vi "takeuchi_2026_01.vi"() -> ()   [LabVIEW 2026]
uses:
  <vilib>/Utility/file.llb/Write Delimited Spreadsheet (DBL).vi
panel:
  out "SOV?":string
  out "Specified voltage":string
  in  "Boolean":bool
  in  "delay time (s)":dbl
  out "Remaining time (s)":i32
  out "XY Graph":cluster{dbl[], dbl[]}(graph)
  in  "Start Voltage(V)":dbl
  in  "Goal Voltage(V)":dbl
  in  "Step (mV)":dbl
  in  "base path":path
  in  "File name":string
  # "temp"
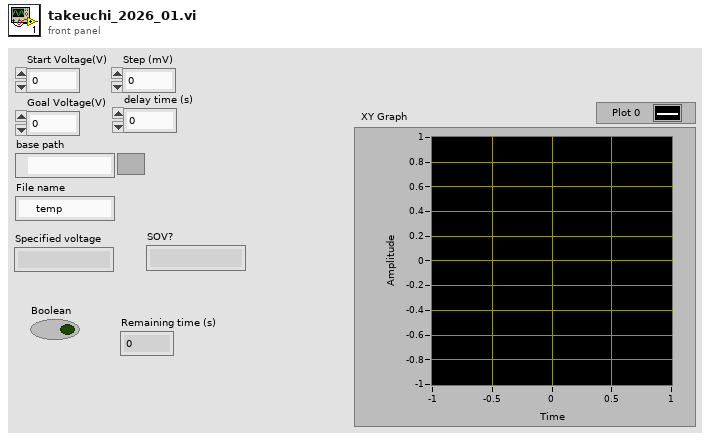
[diagram p1: front panel]
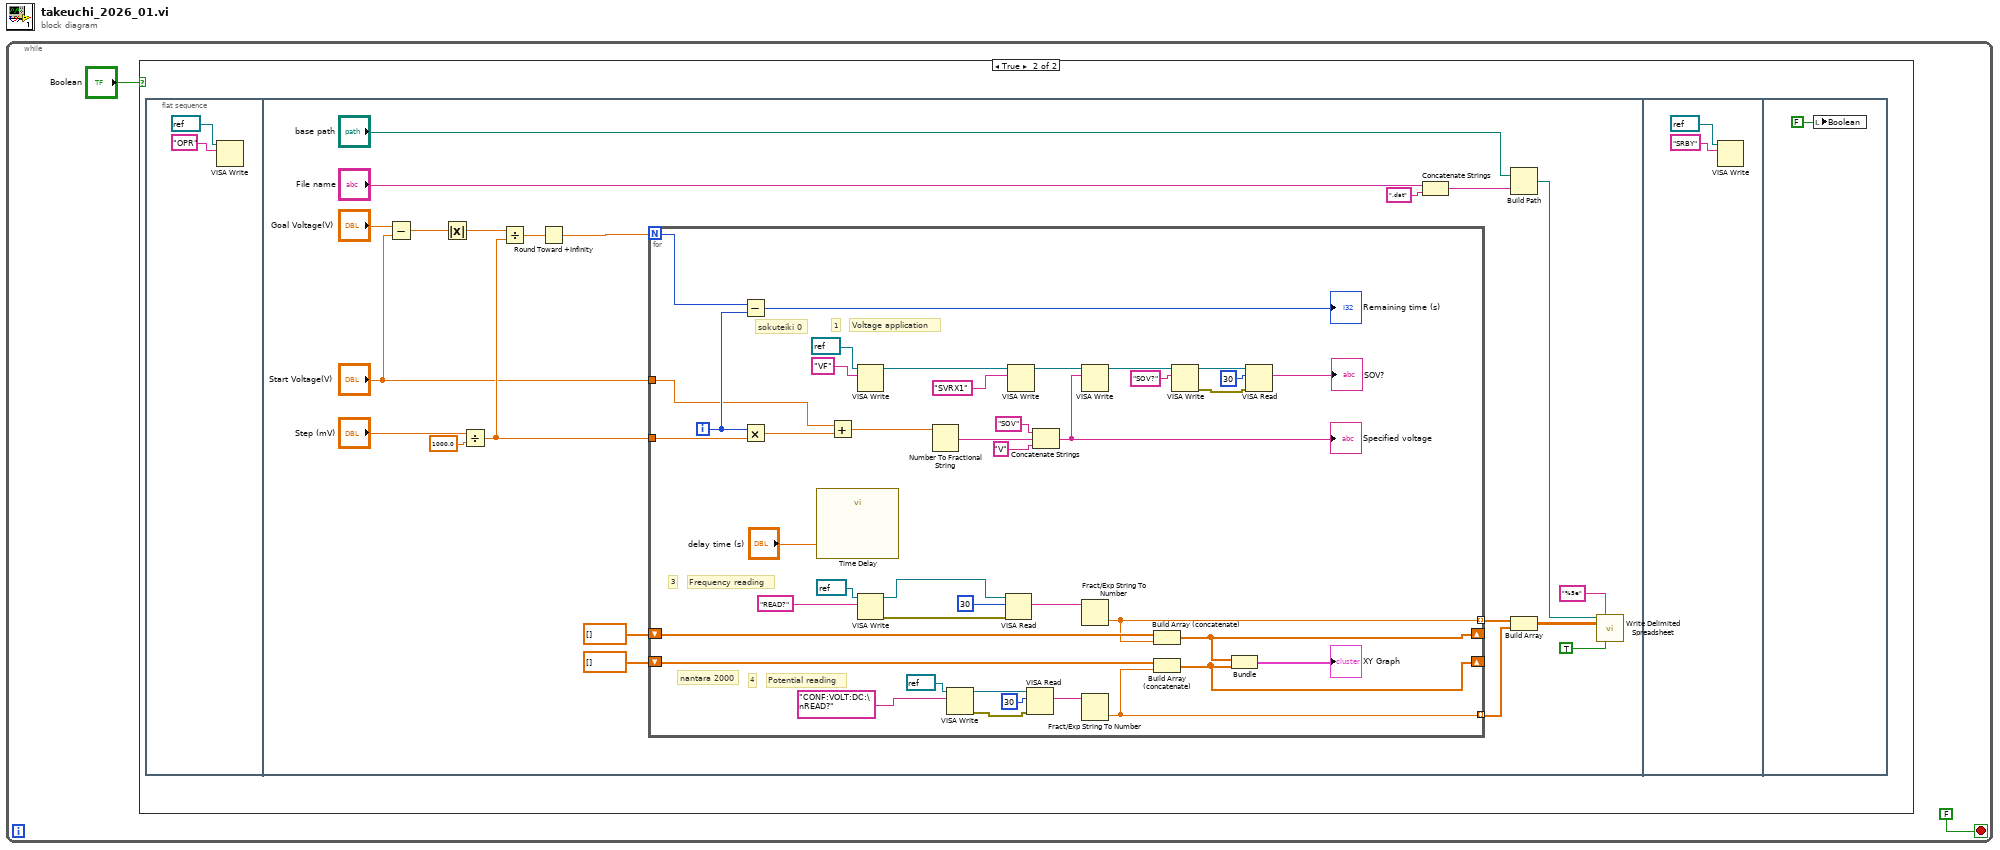
[diagram p0: block diagram]
diagram:
  n1 = while {
    stop <- FALSE stop-if-true
    n2 = case shown="True" "Boolean" {
      frame False {
      }
      frame True {
        n3 = flat-sequence {
          frame #0 {
            n4 = VISA Write(VISA resource name=refnum<visa-resource-name> refnum, write buffer="OPR") -> ()  [unwired: 1 in, 3 out]
          }
          frame #1 {
            n5 = Subtract(x="Goal Voltage(V)", y="Start Voltage(V)") -> (x-y=w24:dbl)
            n6 = Absolute Value(x=w24) -> (abs(x)=w23:dbl)
            n7 = Divide(x="Step (mV)", y=1000.0) -> (x/y=w18:dbl)
            n8 = Divide(x=w23, y=w18) -> (x/y=w20:dbl)
            n9 = Round Toward +Infinity(x=w20) -> (ceil(x): smallest int >= x=w19:dbl)
            n10 = for {
              N: w19 -> [w67]
              tunnel: w18 -> [w65]
              tunnel: "Start Voltage(V)" -> [w63]
              shift-right: [w44] -> _
              shift-left: dbl[] [] ("Numeric 2") -> [w43]
              shift-right: [w46] -> _
              shift-left: dbl[] [] ("Array") -> [w48]
              tunnel: [w42] -> w14 mode=indexing
              tunnel: [w47] -> w13 mode=indexing
              i -> [w66]
              # "sokuteiki 0"
              # "nantara 2000"
              # "1"
              # "3"
              # "4"
              # "Voltage application"
              # "Potential reading"
              # "Frequency reading"
              n11 = Subtract(x=w67, y=w66) -> (x-y=→"Remaining time (s)":i32)
              n12 = Multiply(x=w66, y=w65) -> (x*y=w64:dbl)
              n13 = call "Time Delay"("Delay Time (s)"="delay time (s)") -> ()  [unwired: 10 in, 1 out]
              n14 = Add(x=w63, y=w64) -> (x+y=w61:dbl)
              n15 = VISA Write(VISA resource name=refnum<visa-resource-name> refnum, write buffer="VF") -> (VISA resource name out=w40:refnum<visa-resource-name>)  [unwired: 1 in, 2 out]
              n16 = VISA Write(VISA resource name=refnum<visa-resource-name> refnum, write buffer="READ?") -> (VISA resource name out=w54:refnum<visa-resource-name>, error out=w52:errorcluster)  [unwired: 1 in, 1 out]
              n17 = Number To Fractional String(number=w61) -> (F-format string=w60:string)  [unwired: 3 in]
              n18 = VISA Write(VISA resource name=refnum<visa-resource-name> refnum, write buffer="CONF:VOLT:DC:\nREAD?") -> (VISA resource name out=w34:refnum<visa-resource-name>, error out=w27:errorcluster)  [unwired: 1 in, 1 out]
              n19 = VISA Read(VISA resource name=w54, byte count=u32 30, error in (no error)=w52) -> (read buffer=w50:string)  [unwired: 3 out]
              n20 = VISA Write(VISA resource name=w40, write buffer="SVRX1") -> (VISA resource name out=w39:refnum<visa-resource-name>)  [unwired: 1 in, 2 out]
              n21 = VISA Read(VISA resource name=w34, byte count=u32 30, error in (no error)=w27) -> (read buffer=w49:string)  [unwired: 3 out]
              n22 = Concatenate Strings("SOV", w60, "V") -> (w36:string)
              "Specified voltage" <- w36
              n23 = VISA Write(VISA resource name=w39, write buffer=w36) -> (VISA resource name out=w32:refnum<visa-resource-name>)  [unwired: 1 in, 2 out]
              n24 = Fract/Exp String To Number(string=w50) -> (number=w42:dbl)  [unwired: 3 in, 1 out]
              n25 = Fract/Exp String To Number(string=w49) -> (number=w47:dbl)  [unwired: 3 in, 1 out]
              n26 = Build Array (concatenate)(w43, w42) -> (w44:dbl[])
              n27 = Build Array (concatenate)(w48, w47) -> (w46:dbl[])
              n28 = VISA Write(VISA resource name=w32, write buffer="SOV?") -> (VISA resource name out=w30:refnum<visa-resource-name>, error out=w26:errorcluster)  [unwired: 1 in, 1 out]
              n29 = Bundle(w44, w46) -> (→"XY Graph":cluster{dbl[], dbl[]})  [unwired: 1 in]
              n30 = VISA Read(VISA resource name=w30, byte count=u32 30, error in (no error)=w26) -> (read buffer=→"SOV?":string)  [unwired: 3 out]
            }
            n31 = Concatenate Strings("File name", ".dat" ("string")) -> (w11:string)
            n32 = Build Path(base path="base path", name or relative path=w11) -> (appended path=w8:path)
            n33 = Build Array(w14, w13) -> (w7:dbl[][])
            n34 = call-poly <vilib>:"Write Delimited Spreadsheet.vi"("file path (dialog if empty)"=w8, "format (%.3f)"="%5e", "2D data"=w7, "transpose? (no:F)"=TRUE) -> ()  [unwired: 10 in, 2 out]
          }
          frame #2 {
            n35 = VISA Write(VISA resource name=refnum<visa-resource-name> refnum, write buffer="SRBY") -> ()  [unwired: 1 in, 3 out]
          }
          frame #3 {
            n36 = local write "Boolean"(FALSE) -> ()
          }
        }
      }
    }
  }
